vi "TP1_interface.vi"() -> ()   [LabVIEW 2012]
uses:
  <vilib>/gmath/NI_Gmath.lvlib
panel:
  out "appended array":dbl[](array[numeric])
  out "Numeric 2":i32
  out "Numeric":dbl
  out "Array 2":dbl[](array[numeric])
  out "Array":dbl[](array[numeric])
  out "mean":dbl format="%0.2f"
  in  "stop":bool
  out "Waveform Chart":dbl(graph)
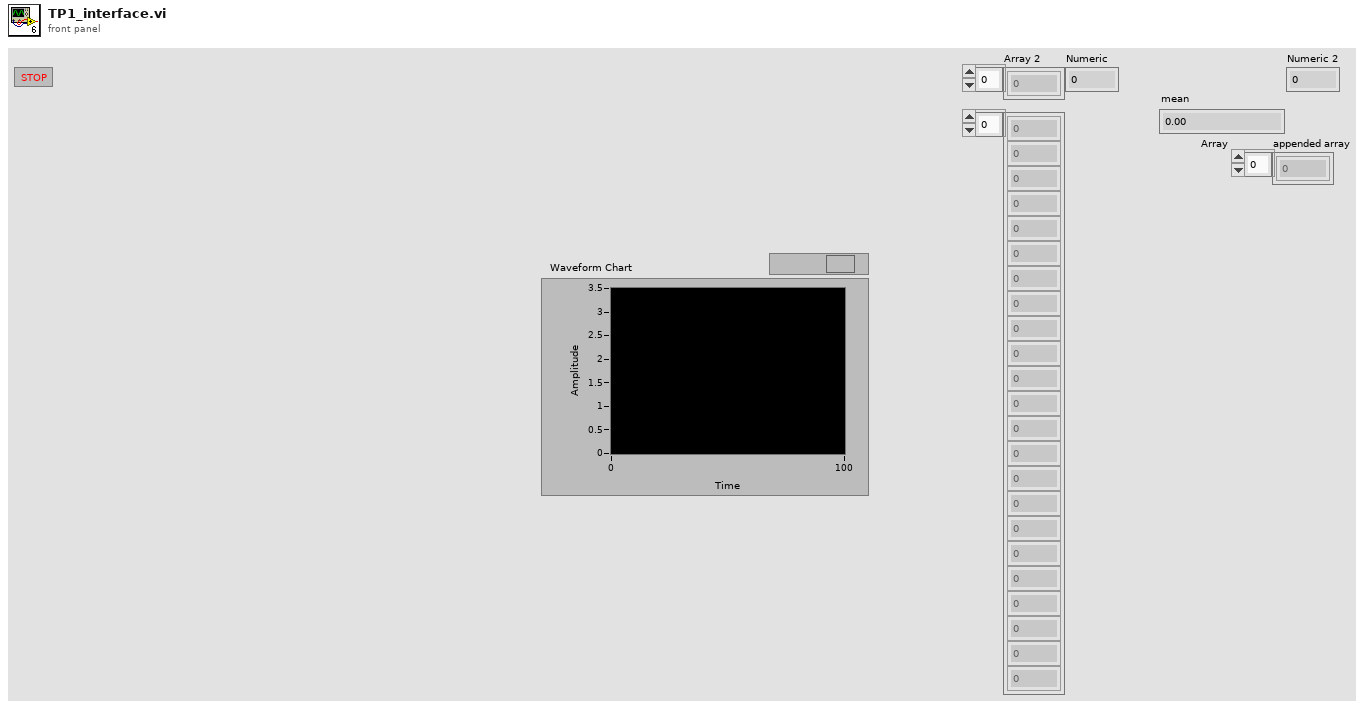
[diagram p1: front panel]
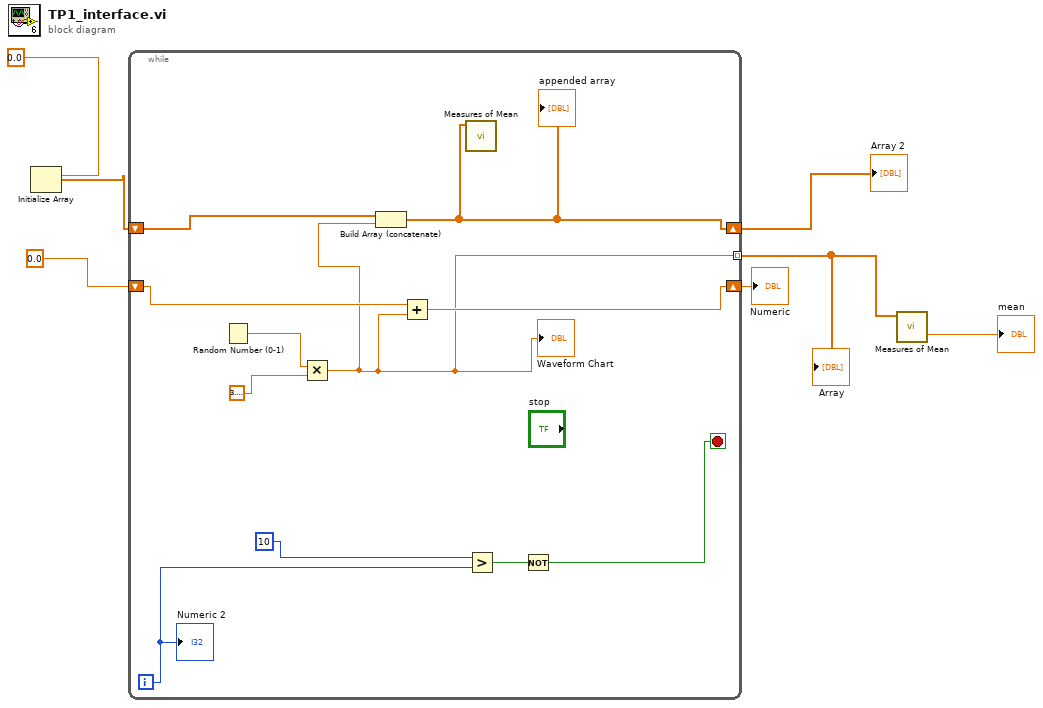
[diagram p0: block diagram]
diagram:
  n1 = Initialize Array(0.0) -> (w4:dbl[])  [unwired: 1 in]
  n2 = while {
    tunnel: [w10] -> w7 mode=indexing
    shift-right: [w8] -> w2
    shift-left: w4 -> [w13]
    shift-right: [w11] -> w1
    shift-left: 0.0 -> [w12]
    i -> [w15]
    stop <- w9 stop-if-true
    n3 = Random Number (0-1)() -> (number: 0 to 1=w18:dbl)
    n4 = Multiply(x=w18, y=3.141592653589793) -> (x*y=w10:dbl)
    "Waveform Chart" <- w10
    n5 = Build Array (concatenate)(w13, w10) -> (w8:dbl[])
    "appended array" <- w8
    n6 = Add(x=w12, y=w10) -> (x+y=w11:dbl)
    n7 = call <vilib>:"Measures of Mean.vi"("x array"=w8) -> ()  [unwired: 9 in, 2 out]
    n8 = Greater?(x=10, y=w15) -> (0:w14:bool)
    n9 = Not(x=w14) -> (.not. x?=w9:bool)
    "Numeric 2" <- w15
  }
  "Array" <- w7
  "Array 2" <- w2
  "Numeric" <- w1
  n10 = call <vilib>:"Measures of Mean.vi"("x array"=w7) -> ("mean value"=→"mean":dbl)  [unwired: 9 in, 1 out]
